vi "Initialize.vi"(8 "error in (no error)":errorcluster, 9 "Reset (True)":bool=TRUE, 10 "ID Query (True)":bool=TRUE, 11 "VISA resource name":refnum<visa-resource-name>) -> (0 "error out":errorcluster, 2 "Identity":T1, 3 "VISA resource name out":refnum<visa-resource-name>)   [LabVIEW 2020, in "HandsOnPi2040.lvlib"]
doc: "Establishes communication with the instrument and optionally performs an instrument identification query and/or an instrument reset. It also places the instrument in a default state needed for other instrument driver operations. Therefore, call this VI before calling other instrument driver VIs for this instrument. Generally, you need to call the <b>Initialize</b> VI only once at the beginning of an application."
uses:
  HandsOnPi2040.lvlib
  cti-drivers-lv-visa-main/CTI-Visa/CTI-Visa.lvlib
  cti-drivers-lv-visa-main/CTI-Visa/Digital Direction.ctl
  cti-drivers-lv-visa-main/CTI-Visa/Identity.ctl
panel:
  # "Input"
  # "Output"
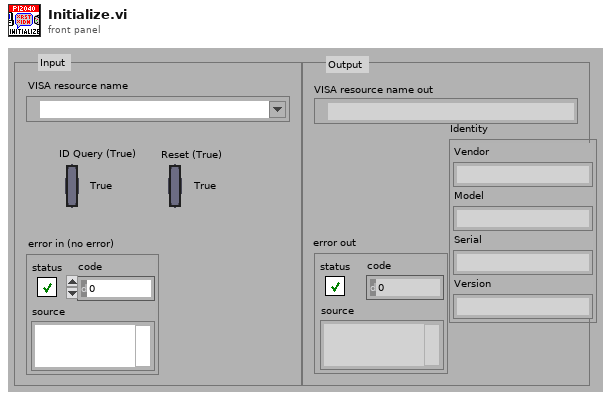
[diagram p1: front panel]
types:
  T1 = typedef "CTI-Visa.lvlib/Identity.ctl" = cluster{"Vendor":string, "Model":string, "Serial":string, "Version":string}
  T2 = typedef "CTI-Visa.lvlib/Digital Direction.ctl" = enum16{"In", "Out"}
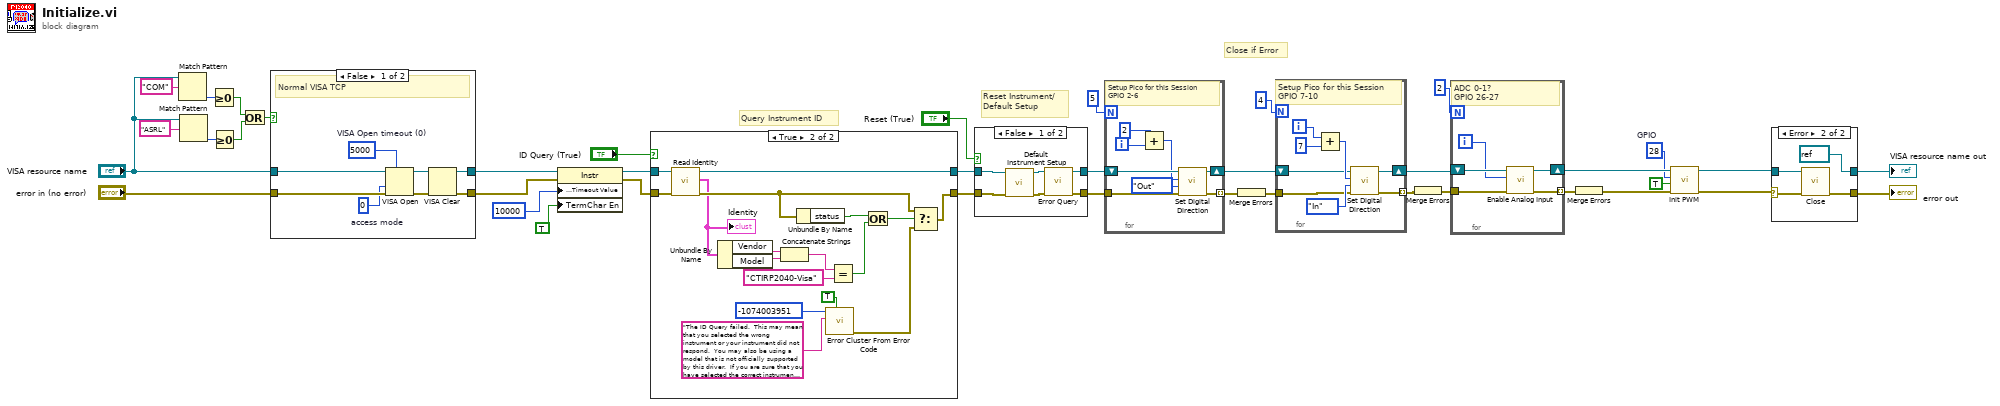
[diagram p0: block diagram]
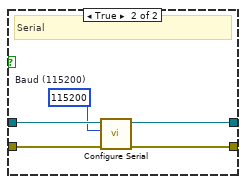
[diagram p2: hidden frame]
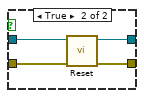
[diagram p4: hidden frame]
diagram:
  w1 = 28  # GPIO
  # "Close if Error"
  # "Query Instrument ID"
  # "Reset Instrument/\nDefault Setup"
  n1 = Match Pattern(string="VISA resource name", regular expression="COM") -> (offset past match=w25:i32)  [unwired: 1 in, 3 out]
  n2 = Match Pattern(string="VISA resource name", regular expression="ASRL") -> (offset past match=w24:i32)  [unwired: 1 in, 3 out]
  n3 = Greater Or Equal To 0?(x=w25) -> (x >= 0?=w23:bool)
  n4 = Greater Or Equal To 0?(x=w24) -> (x >= 0?=w22:bool)
  n5 = Or(x=w23, y=w22) -> (x .or. y?=w21:bool)
  n6 = case shown="False" w21 {
    tunnel: "VISA resource name" -> [w47 w52]
    tunnel: "error in (no error)" -> [w46 w51]
    tunnel: [w41 w50] -> w19
    tunnel: [w40 w49] -> w20
    frame False {
      w44 = u32 5000  # VISA Open timeout (0)
      w45 = u32 0  # access mode
      # "Normal VISA TCP"
      n7 = VISA Open(timeout (0)=w44, access mode=w45, error in (no error)=w46, VISA resource name=w47) -> (VISA resource name=w43:refnum<visa-resource-name>, error out=w42:errorcluster)  [unwired: 1 in]
      n8 = VISA Clear(VISA resource name=w43, error in (no error)=w42) -> (VISA resource name out=w41:refnum<visa-resource-name>, error out=w40:errorcluster)
    }
    frame True {
      w48 = u32 115200  # Baud (115200)
      # "Serial"
      n9 = call "Configure Serial.vi"("error in (no error)"=w51, "Baud (115200)"=w48, "VISA resource name in"=w52) -> ("error out"=w49:errorcluster, "VISA resource name"=w50:refnum<visa-resource-name>)  [unwired: 7 in]
    }
  }
  n10 = property class="Instr"(reference=w19, error in=w20, "General Settings:Timeout Value"=u32 10000, "TermChar En"=TRUE ("Message Based Settings:Termination Character Enable")) -> (reference out=w33:refnum<visa-resource-name>, error out=w32:errorcluster)
  n11 = case shown="True" "ID Query (True)" {
    tunnel: [w53 w71] -> w38
    tunnel: [w54 w64] -> w39
    tunnel: w33 -> [w54 w63]
    tunnel: w32 -> [w53 w62]
    frame False {
    }
    frame True {
      n12 = call "Read Identity.vi"("error in (no error)"=w62, "VISA resource name in"=w63) -> ("error out"=w61:errorcluster, "Identity"=w60:T1, "VISA resource name"=w64:refnum<visa-resource-name>)  [unwired: 7 in]
      "Identity" <- w60
      n13 = Unbundle By Name(w60) -> ("Vendor"=w58:string, "Model"=w59:string)
      n14 = Concatenate Strings(w58, w59) -> (w57:string)
      n15 = Unbundle By Name(w61) -> ("status"=w66:bool)
      n16 = call <vilib>:"Error Cluster From Error Code.vi"("show call chain? (False)"=TRUE, "error message (\"\")"="The ID Query failed.  This may mean that you selected the wrong instrument or your instrument did not respond.  You may also be using a model that is not officially supported by this driver.  If you are sure that you have selected the correct instrument and it is responding, try disabling the ID Query." ("Source (VI Name)"), "error code (0)"=-1074003951 ("Code")) -> ("error out"=w70:errorcluster)  [unwired: 6 in]
      n17 = Equal?(x=w57, y="CTIRP2040-Visa") -> (x = y?=w55:bool)
      n18 = Or(x=w66, y=w55) -> (x .or. y?=w65:bool)
      n19 = Select(t=w61, s=w65, f=w70) -> (s? t:f=w71:errorcluster)
    }
  }
  n20 = case shown="False" "Reset (True)" {
    tunnel: w38 -> [w76 w78]
    tunnel: [w73 w81] -> w17
    tunnel: w39 -> [w77 w79]
    tunnel: [w74 w80] -> w18
    frame False {
      n21 = call "Default Instrument Setup.vi"("error in (no error)"=w76, "VISA resource name"=w77) -> ("error out"=w72:errorcluster, "VISA resource name out"=w75:refnum<visa-resource-name>)  [unwired: 8 in]
      n22 = call "Error Query.vi"("error in (no error)"=w72, "VISA resource name"=w75) -> ("error out"=w73:errorcluster, "VISA resource name out"=w74:refnum<visa-resource-name>)  [unwired: 6 in, 2 out]
    }
    frame True {
      n23 = call "Reset.vi"("error in (no error)"=w78, "VISA resource name"=w79) -> ("error out"=w81:errorcluster, "VISA resource name out"=w80:refnum<visa-resource-name>)  [unwired: 8 in]
    }
  }
  n24 = for {
    N: 5 -> [_]
    shift-right: [w86] -> w9
    shift-left: w18 -> [w89]
    tunnel: w17 -> [w88]
    tunnel: [w85] -> w16 mode=indexing
    i -> [w84]
    # "Setup Pico for this Session\nGPIO 2-6"
    n25 = Add(x=2, y=w84) -> (x+y=w82:i32)
    n26 = call "Set Digital Direction.vi"("error in (no error)"=w88, "Direction"=Digital_Direction."Out", "Channel"=w82, "VISA resource name in"=w89) -> ("error out"=w85:errorcluster, "VISA resource name"=w86:refnum<visa-resource-name>)  [unwired: 6 in]
  }
  n27 = Merge Errors(w16) -> (w10:errorcluster)
  n28 = for {
    N: 4 -> [_]
    shift-right: [w94] -> w8
    shift-left: w9 -> [w91]
    tunnel: [w93] -> w11 mode=indexing
    tunnel: w10 -> [w90]
    i -> [w92]
    # "Setup Pico for this Session\nGPIO 7-10"
    n29 = Add(x=w92, y=7) -> (x+y=w95:i32)
    n30 = call "Set Digital Direction.vi"("error in (no error)"=w90, "Direction"=Digital_Direction."In", "Channel"=w95, "VISA resource name in"=w91) -> ("error out"=w93:errorcluster, "VISA resource name"=w94:refnum<visa-resource-name>)  [unwired: 6 in]
  }
  n31 = Merge Errors(w11) -> (w12:errorcluster)
  n32 = for {
    N: 2 -> [_]
    shift-right: [w100] -> w6
    shift-left: w8 -> [w101]
    tunnel: w12 -> [w102]
    tunnel: [w99] -> w14 mode=indexing
    i -> [w98]
    # "ADC 0-1?\nGPIO 26-27"
    n33 = call "Enable Analog Input.vi"("error in (no error)"=w102, "Channel"=w98, "VISA resource name in"=w101) -> ("error out"=w99:errorcluster, "VISA resource name"=w100:refnum<visa-resource-name>)  [unwired: 7 in]
  }
  n34 = Merge Errors(w14) -> (w5:errorcluster)
  n35 = call "Init PWM.vi"("error in (no error)"=w5, "Enable (F)"=TRUE, "Channel"=w1, "VISA resource name in"=w6) -> ("error out"=w4:errorcluster, "VISA resource name"=w3:refnum<visa-resource-name>)  [unwired: 6 in]
  n36 = case shown="Error" w4 {
    selector: w4 -> [w103 w106]
    tunnel: w3 -> [w104 w107]
    tunnel: [w104 refnum<visa-resource-name> refnum ("VISA resource name out")] -> w31
    tunnel: [w103 w108] -> w30
    frame No Error {
    }
    frame Error {
      n37 = call "Close.vi"("error in (no error)"=w106, "VISA resource name"=w107) -> ("error out"=w108:errorcluster)  [unwired: 9 in]
    }
  }
  "VISA resource name out" <- w31
  "error out" <- w30
